vi "ClassRelationshipEdge_Create.vi"(0 "reference":refnum<class "ClassRelationshipEdge.lvclass">, 5 "error in (no error)":errorcluster) -> (14 "reference out":refnum<class "ClassRelationshipEdge.lvclass">, 19 "error out":errorcluster)   [LabVIEW 2020, in "ClassRelationshipEdge.lvclass"]
doc: "Creates and initializes a new ClassRelationshipEdge object.\n\nThis object should be destroyed using a ClassRelationshipEdge destructor VI or a virtual base class destructor VI.\n\n[GOOP 2.1]"
uses:
  <resource>/Framework/Providers/Open_GDS/UML/ClassRelationshipEdge_class/ClassRelationshipEdge.lvclass
  C:/Program Files (x86)/National Instruments/LabVIEW 2020/resource/Framework/Providers/Open_GDS/UML/SegmentedLineEdge_class/SegmentedLineEdge.lvclass
  <resource>/Framework/Providers/Open_GDS/UML/BentStyle_class/BentStyleType.ctl
  <resource>/Framework/Providers/Open_GDS/UML/SegmentedLineEdge_class/SegmentedLineEdge.lvclass
  <resource>/Framework/Providers/Open_GDS/UML/BentStyle_class/BentStyle.lvclass
panel:
  # "The input reference should only\nbe wired when this method is called\nby a sub class constructor."
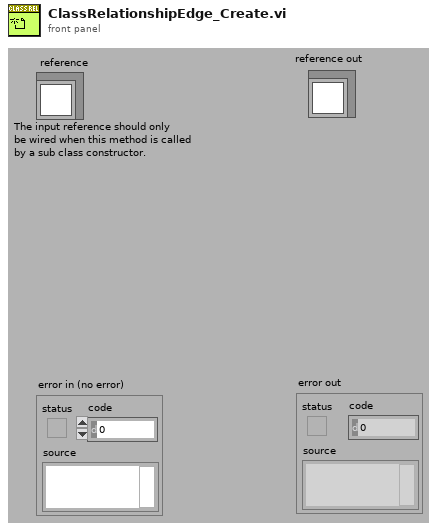
[diagram p1: front panel]
types:
  T1 = typedef "BentStyle.lvclass/BentStyleType.ctl" = enum16{"STRAIGHT", "HV", "VH", "HVH", "VHV", "ARC"}
  T2 = typedef "ClassRelationshipEdge.lvclass/ObjectAttributes.ctl" = cluster{"bentStyleRef":refnum<class "BentStyle.lvclass">, "startConnectionOffset":cluster{"x":i32, "y":i32}, "endConnectionOffset":cluster{"x":i32, "y":i32}, "MidLineOffset":cluster{"x":i32, "y":i32}, "DepClass":T3}
  T3 = typedef "ReversedEngineering_ViDependencyDetailsType.ctl" = cluster{"ThisVIs/Ctls":path[], "Dependent_VIs/Ctls":path[]}
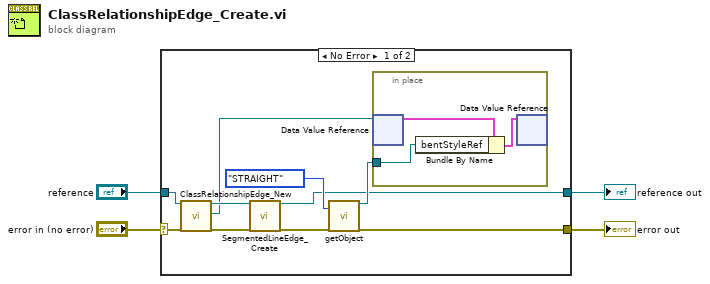
[diagram p0: block diagram]
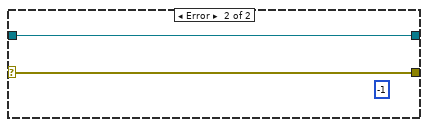
[diagram p2: hidden frame]
diagram:
  n1 = case shown="No Error" "error in (no error)" {
    selector: "error in (no error)" -> [w14 w19]
    tunnel: [w7 w18] -> w4
    tunnel: [w6 w19] -> w3
    tunnel: "reference" -> [w13 w18]
    frame No Error {
      n2 = call <resource>:"ClassRelationshipEdge_New.vi"("reference in"=w13, "error in (no error)"=w14) -> ("reference out"=w11:refnum<class "ClassRelationshipEdge.lvclass">, "DVRRefOut"=w5:refnum<data-value>, "error out"=w12:errorcluster)  [unwired: 2 in, 13 out]
      n3 = call <resource>:"SegmentedLineEdge_Create.vi"("reference"=w11, "error in (no error)"=w12) -> ("reference out"=w7:refnum<class "ClassRelationshipEdge.lvclass">, "error out"=w9:errorcluster)  [unwired: 1 in, 15 out]
      n4 = call <resource>:"getObject.vi"("bentStyle"=BentStyleType."STRAIGHT", "error in (no error)"=w9) -> ("reference out"=w8:refnum<class "BentStyle.lvclass">, "error out"=w6:errorcluster)  [unwired: 16 out]
      n5 = in-place {
        in-place-border: w8 -> [w16]
        n6 = in-place-dvr #1(w5) -> (w17:T2)  [unwired: 1 out]
        n7 = Bundle By Name(cluster=w17, "bentStyleRef"=w16) -> (w15:T2)
        n8 = in-place-dvr #1(w15) -> ()  [unwired: 2 out]
      }
    }
    frame Error {
      (unwired) -1 ("Nr of open handles")
    }
  }
  "error out" <- w3
  "reference out" <- w4
